vi "from string.vi"(8 "error in":errorcluster, 9 "data":string, 10 "version":string, 11 "Submodule EOL configuration":refnum<class "Submodule EOL configuration.lvclass">) -> (0 "error out":errorcluster, 3 "Submodule EOL configuration out":refnum<class "Submodule EOL configuration.lvclass">)   [LabVIEW 2025, in "Submodule EOL.lvlib" / "Submodule EOL configuration.lvclass"]
doc: "Provides an interface for loading a module configuration from a file or other serialized data source. It is recommended that all children of this class store data in two sets--data required for its own initialization, and any data required for parent initialization--and that each implementation uses the <b>Call Parent Method</b> primitive to de-serialize parent information.Copyright 2017 National Instruments Corporation\n\nLicensed under the Apache License, Version 2.0 (the \"License\"); you may not use this file except in compliance with the License. You may obtain a copy of the License at http://www.apache.org/licenses/LICENSE-2.0\nUnless required by applicable law or agreed to in writing, software distributed under the License is distributed on an \"AS IS\" BASIS, WITHOUT WARRANTIES OR CONDITIONS OF ANY KIND, either express or implied. See the License for the specific language governing permissions and limitations under the License."
uses:
  Submodule EOL configuration.lvclass
  Setting.ctl
  PLC.ctl
  Instrumnet.ctl
  Submodule EOL configuration.lvclass/Submodule EOL configuration.ctl
  Users/Public/Documents/Sandia National Labs/TSS Plugin/CEF.lvlibp/serializable configuration/CEF_serializable configuration.lvclass
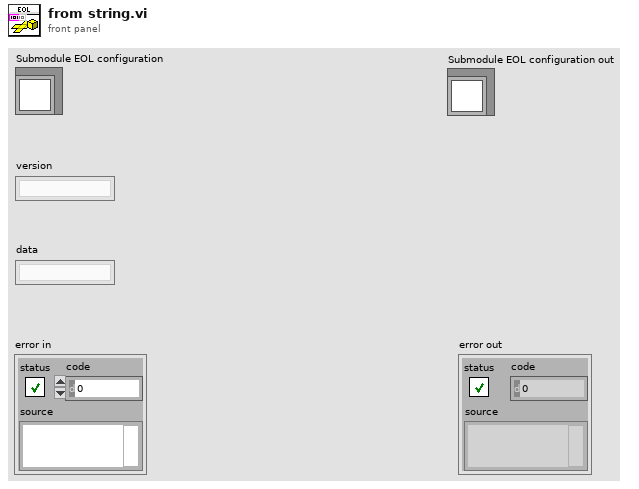
[diagram p1: front panel]
types:
  T1 = typedef "Submodule EOL.lvlib/Submodule EOL configuration.lvclass/Instrumnet.ctl" = cluster{"Digitial IO":string, "HiPOT":string, "ACIR":string, "DMM":string}
  T2 = typedef "Submodule EOL.lvlib/Submodule EOL configuration.lvclass/PLC.ctl" = cluster{"PLC Folder Names":string[][], "PLC URL":string, "Ignition Folder Names":string[][], "Ignition URL":string, "Test Name":string}
  T3 = typedef "Submodule EOL.lvlib/Submodule EOL configuration.lvclass/Setting.ctl" = cluster{"Local Database":string, "Connect OPC Trial":u32, "Timeout Connect OPC":dbl, "AbstractUUT Path":string, "PreUUT Path":string, "Test Path":string, "PostUUT Path":string}
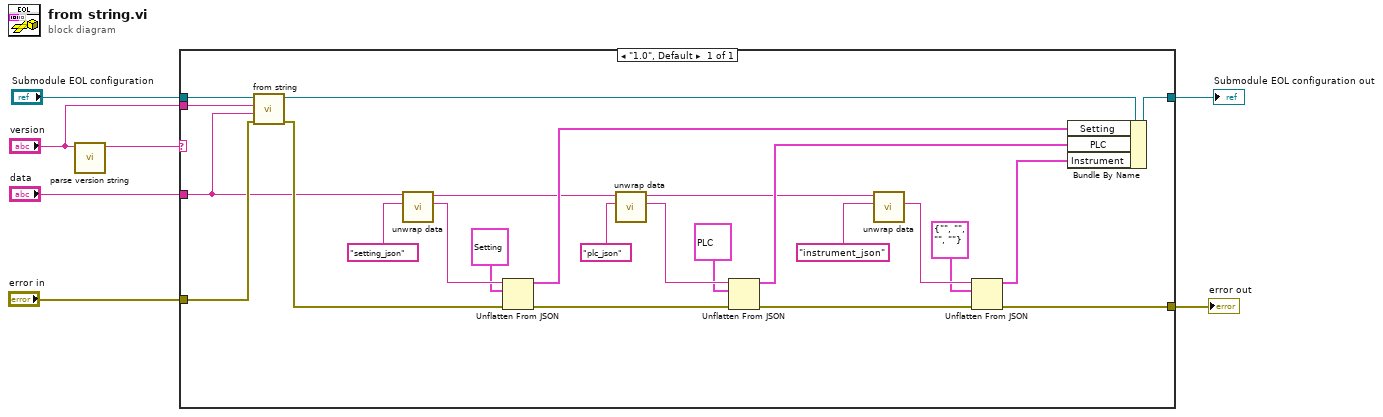
[diagram p0: block diagram]
diagram:
  n1 = call "parse version string.vi"("full version"="version") -> ("major.minor version"=w5:string)  [unwired: 7 in, 3 out]
  n2 = case shown="\"1.0\", Default" w5 {
    tunnel: "Submodule EOL configuration" -> [w31]
    tunnel: [w27] -> w1
    tunnel: "data" -> [w23]
    tunnel: "error in" -> [w29]
    tunnel: [w8] -> w4
    tunnel: "version" -> [w24]
    frame "1.0", Default {
      n3 = call-parent "from string.vi"("error in"=w29, "data"=w23, "version"=w24, "CEF_Configuration in"=w31) -> ("error out"=w28:errorcluster, "CEF_Configuration out"=w30:refnum<class "Submodule EOL configuration.lvclass">)  [unwired: 6 in]
      n4 = call "unwrap data.vi"("identifier"="setting_json" ("additional identifier"), "data to unwrap"=w23) -> ("unwrapped data"=w25:string, "remaining string"=w20:string)  [unwired: 8 in]
      n5 = Unflatten From JSON(JSON string=w25, type and defaults=T3 {"Local Database"="opc.tcp://localhost:49580 ", "Connect OPC Trial"=3, "Timeout Connect OPC"=5.0, "AbstractUUT Path"="opc.tcp://localhost:49580 ", "PreUUT Path"="opc.tcp://10.64.0.22:62541/discovery", "Test Path"="opc.tcp://10.64.0.22:62541/discovery", "PostUUT Path"="Battery Submodule EOL"} ("Event"), error in (no error)=w28) -> (value=w21:T3, error out=w18:errorcluster)  [unwired: 4 in]
      n6 = call "unwrap data.vi"("identifier"="plc_json" ("additional identifier"), "data to unwrap"=w20) -> ("unwrapped data"=w17:string, "remaining string"=w14:string)  [unwired: 8 in]
      n7 = Unflatten From JSON(JSON string=w17, type and defaults=T2 {"PLC Folder Names"=[["Station0_Rx", "OP50A_TesterRxSignals"], ["Station0_Tx", "OP50A_TesterTxSignals"], ["Station1_Rx", "OP50B_TesterRxSignals"], ["Station1_Tx", "OP50B_TesterTxSignals"], ["Station2_Rx", "OP60A_TesterRxSignals"], ["Station2_Tx", "OP60A_TesterTxSignals"], ["Station3_Rx", "OP60B_TesterRxSignals"], ["Station3_Tx", "OP60B_TesterTxSignals"], ["Station4_Rx", "OP70A_TesterRxSignals"], ["Station4_Tx", "OP70A_TesterTxSignals"], ["Station5_Rx", "OP70B_TesterRxSignals"], ["Station5_Tx", "OP70B_TesterTxSignals"]], "PLC URL"="opc.tcp://localhost:49580 ", "Ignition Folder Names"=[["Ignition0_Rx", "[Submodule_EOL]/StaA/TesterRx"], ["Ignition0_Tx", "[Submodule_EOL]/StaA/TesterTx"], ["Ignition1_Rx", "[Submodule_EOL]/StaB/TesterRx"], ["Ignition1_Tx", "[Submodule_EOL]/StaB/TesterTx"], ["Ignition2_Rx", "[Submodule_EOL]/StaC/TesterRx"], ["Ignition2_Tx", "[Submodule_EOL]/StaC/TesterTx"], ["Ignition3_Rx", "[Submodule_EOL]/StaD/TesterRx"], ["Ignition3_Tx", "[Submodule_EOL]/StaD/TesterTx"], ["Ignition4_Rx", "[Submodule_EOL]/StaE/TesterRx"], ["Ignition4_Tx", "[Submodule_EOL]/StaE/TesterTx"], ["Ignition5_Rx", "[Submodule_EOL]/StaF/TesterRx"], ["Ignition5_Tx", "[Submodule_EOL]/StaF/TesterTx"]], "Ignition URL"="opc.tcp://10.64.0.22:62541/discovery", "Test Name"="Battery Submodule EOL"} ("PLC"), error in (no error)=w18) -> (value=w15:T2, error out=w9:errorcluster)  [unwired: 4 in]
      n8 = call "unwrap data.vi"("identifier"="instrument_json" ("additional identifier"), "data to unwrap"=w14) -> ("unwrapped data"=w12:string)  [unwired: 8 in, 1 out]
      n9 = Unflatten From JSON(JSON string=w12, type and defaults=T1 {"Digitial IO"="", "HiPOT"="", "ACIR"="", "DMM"=""} ("Instrument"), error in (no error)=w9) -> (value=w10:T1, error out=w8:errorcluster)  [unwired: 4 in]
      n10 = Bundle By Name(cluster=w30, "Setting"=w21, "PLC"=w15, "Instrument"=w10) -> (w27:refnum<class "Submodule EOL configuration.lvclass">)
    }
  }
  "error out" <- w4
  "Submodule EOL configuration out" <- w1
